vi "Read flow control.vi"(8 "error in (no error)":errorcluster, 11 "Modbus_RTU in":refnum<class "Modbus_RTU.lvclass">) -> (0 "error out":errorcluster, 2 "flow control (none)":u16(ring) items=["None", "XON/XOFF", "RTS/CTS", "XON/XOFF & RTS/CTS", "DTR/DSR", "XON/XOFF & DTR/DSR"], 3 "Modbus_RTU out":refnum<class "Modbus_RTU.lvclass">)   [LabVIEW 2021, in "Modbus_RTU.lvclass"]
uses:
  Modbus_RTU.lvclass
  Modbus_RTU.lvclass/Modbus_RTU.ctl
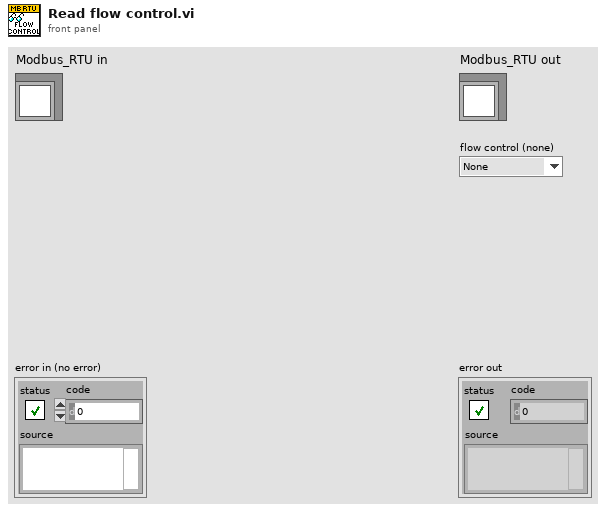
[diagram p1: front panel]
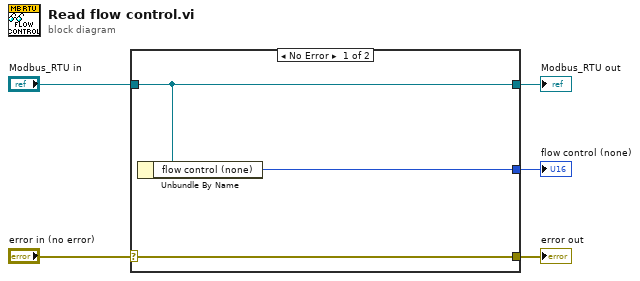
[diagram p0: block diagram]
diagram:
  n1 = case shown="No Error" "error in (no error)" {
    selector: "error in (no error)" -> [w8 w9]
    tunnel: [w8 w9] -> w4
    tunnel: [w7 w10] -> w2
    tunnel: "Modbus_RTU in" -> [w7 w10]
    tunnel: [w6 _] -> w1
    frame No Error {
      n2 = Unbundle By Name(w7) -> ("flow control (none)"=w6:u16)
    }
    frame Error {
    }
  }
  "error out" <- w4
  "Modbus_RTU out" <- w2
  "flow control (none)" <- w1
